vi "Disable Automatic Error Handling.vi"(8 "error in":errorcluster, 11 "VI in":refnum<vi>) -> (0 "error out":errorcluster, 3 "VI out":refnum<vi>)   [LabVIEW 2020, in "MCP Server.lvlib"]
doc: "Switches off LabVIEW's automatic error handling of a tool or prompt VI in memory before the VI is called.\n\nTool and prompt VIs are run with the Run VI method. When such a VI has automatic error handling enabled (the LabVIEW default for new VIs) and an error appears on an output that is not wired, LabVIEW opens its modal error dialog. The call then never returns, and because requests are handled one at a time, the whole MCP server stops answering until someone presses Continue in the LabVIEW IDE.\n\nThe property is read first and written only when it is TRUE, so a VI that already has it off is not marked as modified. The VI is not saved; the change lasts as long as the VI stays in memory. The write is not possible in a built application or while the VI is reserved by a running hierarchy (error 1073); errors of the read and the write are discarded. error in is passed through unchanged."
uses:
  MCP Server.lvlib
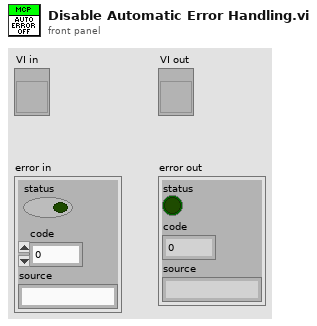
[diagram p1: front panel]
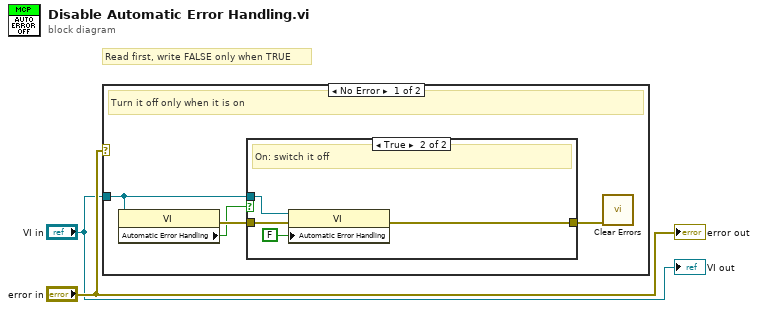
[diagram p0: block diagram]
diagram:
  # "Read first, write FALSE only when TRUE"
  n1 = case shown="No Error" "error in" {
    tunnel: "VI in" -> [w3 _]
    frame No Error {
      # "Turn it off only when it is on"
      n2 = property class="VI"(reference=w3) -> (error out=w5:errorcluster, "Automatic Error Handling"=w4:bool)  [unwired: 1 in, 1 out]
      n3 = case shown="True" w4 {
        tunnel: w3 -> [_ w8]
        tunnel: w5 -> [w7 w9]
        tunnel: [w7 w11] -> w6
        frame False {
          # "Already off: leave it"
        }
        frame True {
          # "On: switch it off"
          n4 = property class="VI"(reference=w8, error in=w9, "Automatic Error Handling"=FALSE) -> (error out=w11:errorcluster)  [unwired: 1 out]
        }
      }
      n5 = call <vilib>:"Clear Errors.vi"("error in (no error)"=w6) -> ()  [unwired: 5 in, 2 out]
    }
    frame Error {
      # "An error came in: do nothing"
    }
  }
  "VI out" <- "VI in"
  "error out" <- "error in"
